vi "VHistFile - Save newest history data.vi"(6 "file params":T2={"path pattern"=enum."Y\\M\\D\\Tag.ext", "file extension (.bin)"=".bin"}, 7 "VC Handle":T1=-1, 8 "error in":errorcluster, 9 "log directory":path=path "DataLog", 10 "file tag":string, 11 "name_spec":string) -> (0 "error out":errorcluster, 2 "dup file tag":string, 3 "dup name_spec":string, 5 "dup VC Handle":T1=-1)   [LabVIEW 2021]
doc: "The VI acquires the newest history data for the specified variable and writes the data to log file(s) in accordance with the specified parameters: <b>file tag</b>, <b>log directory</b> and <b>file params</b>. The VI recognises a variable datatype and saves data in an appropriate format. If a variable has a datatype that the VI does not support, it saves variable values in the Flattened-To-String format.\n\n<B>VC Handle</B> and <B>name_spec</B> controls specify a desired variable.\n\n<b>VC Handle</b> control has to contain a handle of variable context if <b>name_spec</b> control contains a variable name. In order to refer to a global variable, pass -1 to it. <b>VC Handle</b> is ignored if <b>name_spec</b> refers to a variable by alias.\n\n<b>name_spec</b> control has to contain a name specifier referring to a desired variable. Generic format of a name specifier is\n [name][=alias]\n, where\n 'name' is a variable name.\n 'alias' is an alias associated with a variable; it must follow equal sign (=).\nEither 'name' or '=alias' may be omitted but not both.\n\n::: CalcExpress Toolkit :::\nCopyright (c) 2000-2026 Konstantin Shifershteyn. All rights reserved."
uses:
  cetypes.llb/VarMan Variable Context Handle.ctl
  cetypes.llb/CalcExpress Data Type.ctl
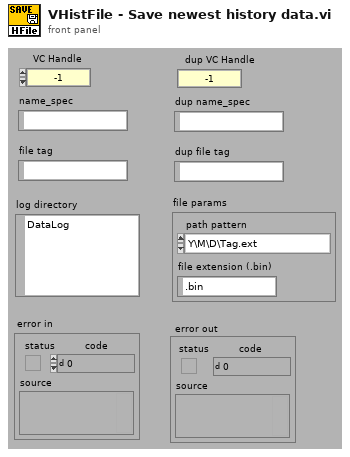
[diagram p1: front panel]
types:
  T1 = typedef "VarMan Variable Context Handle.ctl" = i32
  T2 = cluster{"path pattern":enum32{"Y\\M\\D\\Tag.ext", "Y\\M\\D\\Tag [Y-M-D].ext", "Y-M-D\\Tag.ext", "Y-M-D\\Tag [Y-M-D].ext", "Tag [Y-M-D].ext"}, "file extension (.bin)":string}
  T3 = typedef "VarMan History Info.ctl" = cluster{"var type":u32, "history length":u32, "stored values":u32, "update cnt":u32, "last update ms":u32, "newest timestamp":dbl, "oldest timestamp":dbl, "NewVals mode":cluster{"NewVals cnt":u32, "last read time":dbl, "last read ms":u32}, "time condition":cluster{"Step, ms":u32, "Gate, ms":u32}, "value condition":cluster{"condition":enum32{"don't test", "changed", "abs deviation", "rel deviation", "out of range", "within range"}, "Delta":dbl, "Range_Min":dbl, "Range_Max":dbl}}
  T4 = typedef "CalcExpress Data Type.ctl" = enum32{"String", "DBL Number", "identifier", "1D Array of DBL", "2D Array of DBL", "CDB Number", "1D Array of CDB", "2D Array of CDB", "1D Array of String", "2D Array of String", "Unknown data type"}
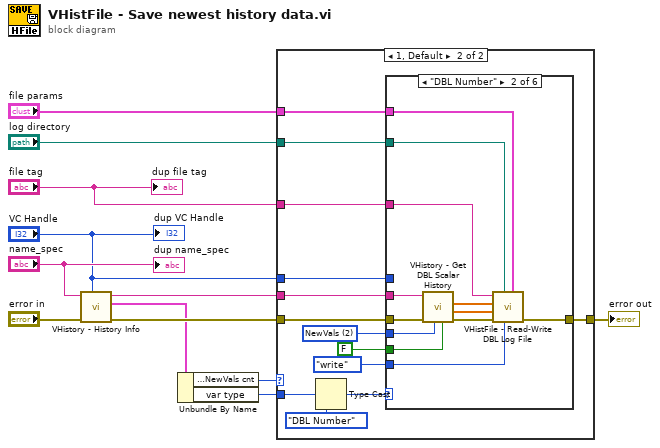
[diagram p0: block diagram]
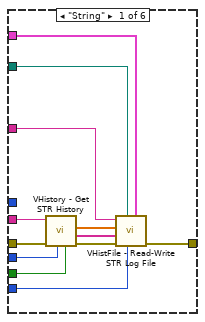
[diagram p3: hidden frame]
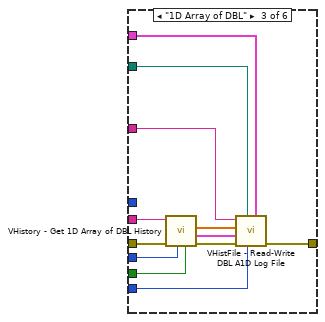
[diagram p4: hidden frame]
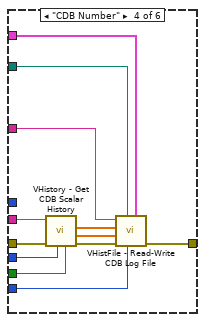
[diagram p5: hidden frame]
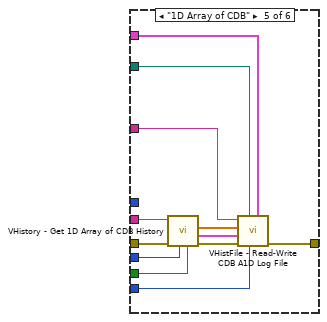
[diagram p6: hidden frame]
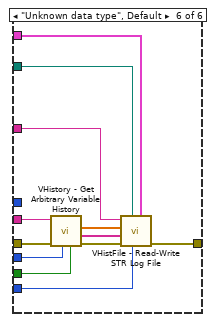
[diagram p7: hidden frame]
diagram:
  n1 = call "VHistory - History Info.vi"("VC Handle"="VC Handle", "error in"="error in", "name_spec"="name_spec") -> ("error out"=w12:errorcluster, "history info"=w10:T3, "dup name_spec"=w9:string)  [unwired: 4 in, 2 out]
  n2 = Unbundle By Name(w10) -> ("NewVals mode.NewVals cnt"=w11:u32, "var type"=w6:u32)
  n3 = case shown="1, Default" w11 {
    tunnel: w12 -> [w13 w26]
    tunnel: w9 -> [_ w21]
    tunnel: [w13 w25] -> w7
    tunnel: w6 -> [_ w23]
    tunnel: "file tag" -> [_ w20]
    tunnel: "VC Handle" -> [_ w19]
    tunnel: "log directory" -> [_ w15]
    tunnel: "file params" -> [_ w14]
    frame 0 {
    }
    frame 1, Default {
      w18 = u32 2 items=["TimeRange", "N-Vals", "NewVals"] ("mode")
      n4 = Type Cast(type=CalcExpress_Data_Type."DBL Number" ("data type"), x=w23) -> (*(type *) &x=w22:T4)
      n5 = case shown="\"DBL Number\"" w22 {
        tunnel: w26 -> [w35 w47 w59 w71 w83 w95]
        tunnel: w21 -> [w34 w46 w58 w70 w82 w94]
        tunnel: [w33 w45 w57 w69 w81 w93] -> w25
        tunnel: w15 -> [w32 w44 w56 w68 w80 w92]
        tunnel: w14 -> [w31 w43 w55 w67 w79 w91]
        tunnel: w20 -> [w30 w42 w54 w66 w78 w90]
        tunnel: w19 -> [_ _ _ _ _ _]
        tunnel: w18 -> [w29 w41 w53 w65 w77 w89]
        tunnel: FALSE ("reverse order (T)") -> [w28 w40 w52 w64 w76 w88]
        tunnel: enum16{"nop", "read", "write", "retrieve"}."write" ("operation") -> [w27 w39 w51 w63 w75 w87]
        frame "String" {
          n6 = call "VHistory - Get STR History.vi"("reverse order (T)"=w28, "mode"=w29, "error in"=w35, "name_spec"=w34) -> ("error out"=w38:errorcluster, "history"=w36:string[], "time stamps"=w37:dbl[])  [unwired: 3 in, 2 out]
          n7 = call "VHistFile - Read-Write STR Log File.vi"("file params"=w31, "operation"=w27, "log directory"=w32, "error in"=w38, "history data in"=w36, "time stamps in"=w37, "file tag"=w30) -> ("error out"=w33:errorcluster)  [unwired: 2 in, 2 out]
        }
        frame "DBL Number" {
          n8 = call "VHistory - Get DBL Scalar History.vi"("reverse order (T)"=w40, "mode"=w41, "error in"=w47, "name_spec"=w46) -> ("error out"=w50:errorcluster, "history"=w48:dbl[], "time stamps"=w49:dbl[])  [unwired: 3 in, 2 out]
          n9 = call "VHistFile - Read-Write DBL Log File.vi"("file params"=w43, "operation"=w39, "log directory"=w44, "error in"=w50, "history data in"=w48, "time stamps in"=w49, "file tag"=w42) -> ("error out"=w45:errorcluster)  [unwired: 2 in, 2 out]
        }
        frame "1D Array of DBL" {
          n10 = call "VHistory - Get 1D Array of DBL History.vi"("reverse order (T)"=w52, "mode"=w53, "error in"=w59, "name_spec"=w58) -> ("error out"=w62:errorcluster, "history"=w60:cluster{"data":dbl[]}[], "time stamps"=w61:dbl[])  [unwired: 3 in, 2 out]
          n11 = call "VHistFile - Read-Write DBL A1D Log File.vi"("file params"=w55, "operation"=w51, "log directory"=w56, "error in"=w62, "history data in"=w60, "time stamps in"=w61, "file tag"=w54) -> ("error out"=w57:errorcluster)  [unwired: 2 in, 2 out]
        }
        frame "CDB Number" {
          n12 = call "VHistory - Get CDB Scalar History.vi"("reverse order (T)"=w64, "mode"=w65, "error in"=w71, "name_spec"=w70) -> ("error out"=w74:errorcluster, "history"=w72:cdb[], "time stamps"=w73:dbl[])  [unwired: 3 in, 2 out]
          n13 = call "VHistFile - Read-Write CDB Log File.vi"("file params"=w67, "operation"=w63, "log directory"=w68, "error in"=w74, "history data in"=w72, "time stamps in"=w73, "file tag"=w66) -> ("error out"=w69:errorcluster)  [unwired: 2 in, 2 out]
        }
        frame "1D Array of CDB" {
          n14 = call "VHistory - Get 1D Array of CDB History.vi"("reverse order (T)"=w76, "mode"=w77, "error in"=w83, "name_spec"=w82) -> ("error out"=w86:errorcluster, "history"=w84:cluster{"data":cdb[]}[], "time stamps"=w85:dbl[])  [unwired: 3 in, 2 out]
          n15 = call "VHistFile - Read-Write CDB A1D Log File.vi"("file params"=w79, "operation"=w75, "log directory"=w80, "error in"=w86, "history data in"=w84, "time stamps in"=w85, "file tag"=w78) -> ("error out"=w81:errorcluster)  [unwired: 2 in, 2 out]
        }
        frame "Unknown data type", Default {
          n16 = call "VHistory - Get Arbitrary Variable History.vi"("reverse order (T)"=w88, "mode"=w89, "error in"=w95, "name_spec"=w94) -> ("error out"=w98:errorcluster, "history"=w96:string[], "time stamps"=w97:dbl[])  [unwired: 3 in, 2 out]
          n17 = call "VHistFile - Read-Write STR Log File.vi"("file params"=w91, "operation"=w87, "log directory"=w92, "error in"=w98, "history data in"=w96, "time stamps in"=w97, "file tag"=w90) -> ("error out"=w93:errorcluster)  [unwired: 2 in, 2 out]
        }
      }
    }
  }
  "error out" <- w7
  "dup file tag" <- "file tag"
  "dup name_spec" <- "name_spec"
  "dup VC Handle" <- "VC Handle"
